vi "[ce] Eval y=f(a,x).vi"(5 "include end point":bool, 6 "parameters":cluster{"name":string, "value":dbl}[](array[cluster]) {"value" format="%.2f"}, 7 "# points":u32=100, 8 "error in":errorcluster, 9 "formula info":cluster{"formula":string, "x-variable":string}={"formula"="", "x-variable"="t"}, 10 "end":dbl=1.0 format="%.2f", 11 "start":dbl format="%.2f") -> (0 "error out":errorcluster, 2 "Y Values":dbl[](array[numeric]) format="%.2f", 3 "X Values":dbl[](array[numeric]) format="%.2f", 4 "ticks":u32)   [LabVIEW 2021]
doc: "Calculates values of the given 1D function. In addition, the VI allows specifying additional parameters and evaluating them in formula.\n\n::: CalcExpress Toolkit :::\nCopyright (c) 2000-2026 Konstantin Shifershteyn. All rights reserved."
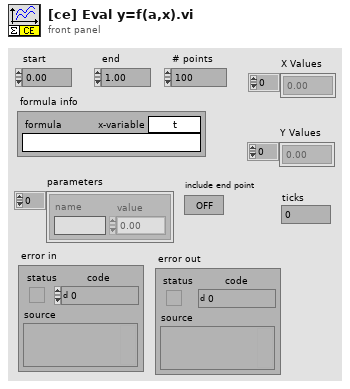
[diagram p1: front panel]
types:
  T1 = enum16{"create", "destroy", "set value", "get value"}
  T2 = typedef "VarMan Variable Context Handle.ctl" = i32
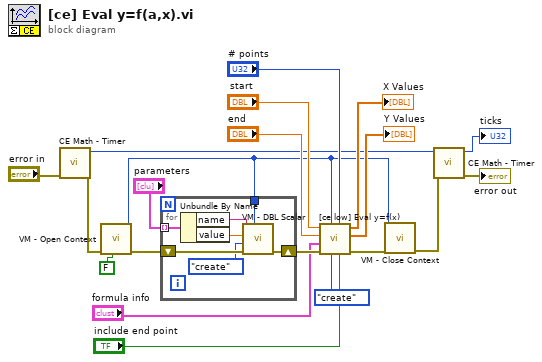
[diagram p0: block diagram]
diagram:
  n1 = call "CE Math - Timer.vi"("error in (no error)"="error in") -> ("error out"=w13:errorcluster, "ticks out"=w14:u32)  [unwired: 7 in]
  n2 = call "VM - Open Context.vi"("close loose contexts (F)"=FALSE ("close loose contexts (T)"), "error in"=w13) -> ("error out"=w8:errorcluster, "VC Handle out"=w2:T2)  [unwired: 7 in, 1 out]
  n3 = for {
    shift-right: [w24] -> w9
    shift-left: w8 -> [w25]
    tunnel: "parameters" -> [w22] mode=indexing
    tunnel: w2 -> [w21]
    n4 = Unbundle By Name(w22) -> ("name"=w26:string, "value"=w27:dbl)
    n5 = call "VM - DBL Scalar.vi"("VC Handle"=w21, "error in"=w25, "cmd"=T1."create", "value in"=w27, "name_spec"=w26) -> ("error out"=w24:errorcluster)  [unwired: 1 in, 5 out]
  }
  n6 = call "[ce low] Eval y=f(x).vi"("include end point"="include end point", "# points"="# points", "vm cmd"=T1."create", "VC Handle"=w2, "error in"=w9, "formula info"="formula info", "end"="end", "start"="start") -> ("error out"=w20:errorcluster, "f(x)"=→"Y Values":dbl[], "x"=→"X Values":dbl[])  [unwired: 1 out]
  n7 = call "VM - Close Context.vi"("error in"=w20, "VC Handle"=w2) -> ("error out"=w11:errorcluster)  [unwired: 8 in, 1 out]
  n8 = call "CE Math - Timer.vi"("error in (no error)"=w11, "ticks in"=w14) -> ("error out"=→"error out":errorcluster, "ticks out"=→"ticks":u32)  [unwired: 6 in]
